vi "MecaKinematics_ToChassisSpeeds.vi"(9 "MECA_WHEEL_SPEEDS":T4 {"RearRightSpeed" format="%19.3f"; "RearLeftSpeed" format="%19.3f"; "FrontRightSpeed" format="%19.3f"; "FrontLeftSpeed" format="%19.3f"}, 11 "in MECA_DRIVE_KINEMATICS":T1={"FrontLeft"={"X"=0.0, "Y"=0.0}, "FrontRight"={"X"=0.0, "Y"=0.0}, "RearLeft"={"X"=0.0, "Y"=0.0}, "RearRight"={"X"=0.0, "Y"=0.0}, "InverseKinematics"=[[0.0, 1.0, -1.0, 0.0], [0.0, 1.0, 1.0, 0.0], [0.0, 1.0, 1.0, 0.0], [0.0, 1.0, -1.0, 0.0]], "ForwardKinematics"=[[0.0, 1.0, -1.0, 0.0], [0.0, 1.0, 1.0, 0.0], [0.0, 1.0, 1.0, 0.0], [0.0, 1.0, -1.0, 0.0]], "PrevCoR"={"X"=0.0, "Y"=0.0}} {"PrevCoR"."Y" format="%14.3f"; "PrevCoR"."X" format="%14.3f"; "RearRight"."Y" format="%14.3f"; "RearRight"."X" format="%14.3f"; "RearLeft"."Y" format="%14.3f"; "RearLeft"."X" format="%14.3f"; "FrontRight"."Y" format="%14.3f"; "FrontRight"."X" format="%14.3f"; "FrontLeft"."Y" format="%14.3f"; "FrontLeft"."X" format="%14.3f"}) -> (3 "ChassisSpeeds":T5 {"vOmega" format="%10.3f"; "vY" format="%10.3f"; "vX" format="%10.3f"})   [LabVIEW 2019, in "Trajectory_Library.lvlib"]
doc: "Performs forward kinematics to return the resulting chassis state from the given wheel speeds. This method is often used for odometry -- determining the robot's position on the field using data from the real-world speed of each wheel on the robot.\n\nParametetrs:\n - MecaDriveKinematics - Data structure\n - WheelSpeeds - The current mecanum drive wheel speeds.\n\nReturns:\n - ChassisSpeeds - The resulting chassis speed."
uses:
  Trajectory_Library.lvlib
  <vilib>/Analysis/Matrix/NI_Matrix.lvlib
  <vilib>/Analysis/Matrix/Numeric/Multiply/Multiply - RM,RM.vi
  TypeDef/TRANSLATION2D.ctl
  TypeDef/CHASSIS_SPEEDS.ctl
  TypeDef/MECA_WHEEL_SPEEDS.ctl
  <vilib>/Analysis/Matrix/Datatypes/RealMatrix.ctl
  TypeDef/MECA_DRIVE_KINEMATICS.ctl
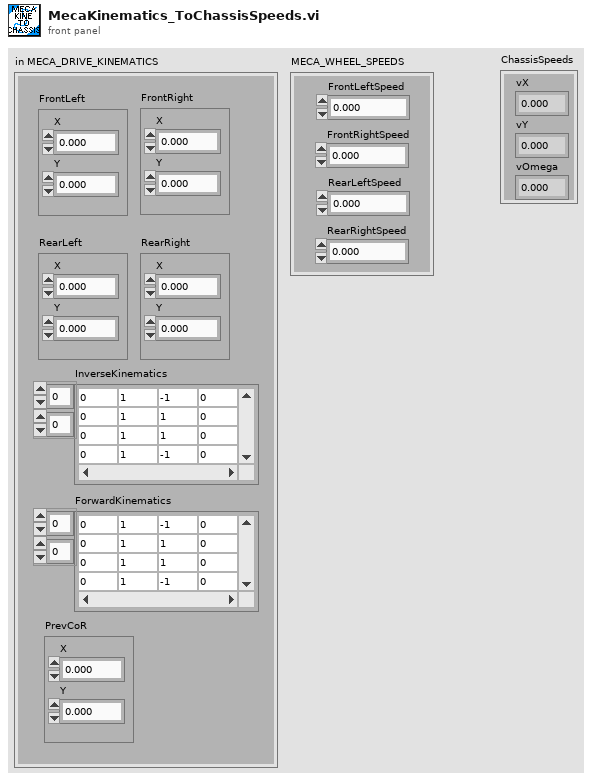
[diagram p1: front panel]
types:
  T1 = typedef "Trajectory_Library.lvlib/MECA_DRIVE_KINEMATICS.ctl" = cluster{"FrontLeft":T2, "FrontRight":T2, "RearLeft":T2, "RearRight":T2, "InverseKinematics":T3, "ForwardKinematics":T3, "PrevCoR":T2}
  T2 = typedef "Trajectory_Library.lvlib/TRANSLATION2D.ctl" = cluster{"X":dbl, "Y":dbl}
  T3 = typedef "NI_Matrix.lvlib/RealMatrix.ctl" = dbl[][]
  T4 = typedef "Trajectory_Library.lvlib/MECA_WHEEL_SPEEDS.ctl" = cluster{"FrontLeftSpeed":dbl, "FrontRightSpeed":dbl, "RearLeftSpeed":dbl, "RearRightSpeed":dbl}
  T5 = typedef "Trajectory_Library.lvlib/CHASSIS_SPEEDS.ctl" = cluster{"vX":dbl, "vY":dbl, "vOmega":dbl}
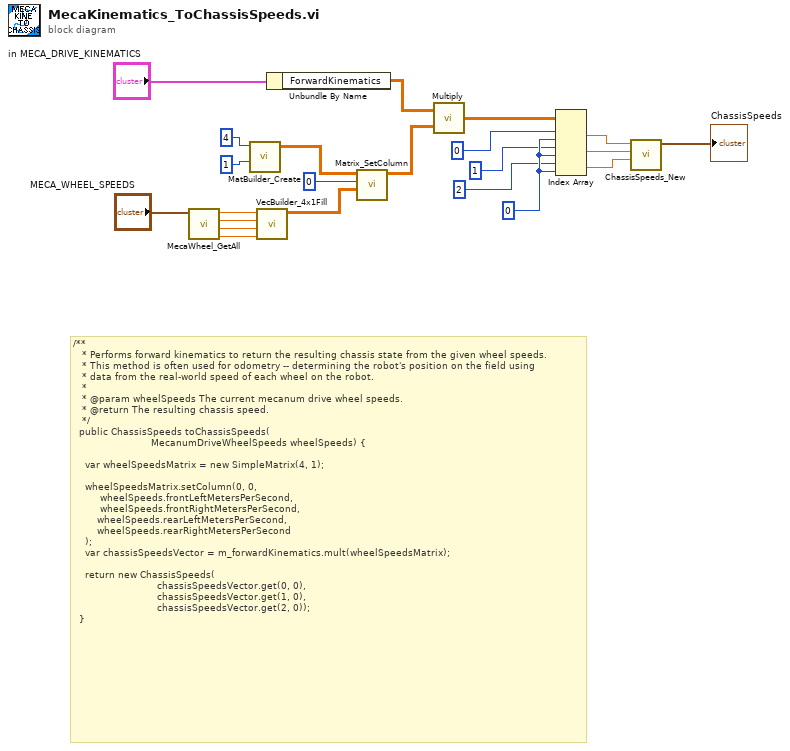
[diagram p0: block diagram]
diagram:
  w22 = 0 ("index (col)")
  # "/**\n   * Performs forward kinematics to return the resulting chassis state from the given wheel speeds.\n   * This method is often used for odometry -- determining the robot's position on the field using\n   * data from the real-world speed of each wheel on the robot.\n   *\n   * @param wheelSpeeds The current mecanum drive wheel speeds.\n   * @return The resulting chassis speed.\n   */\n  public ChassisSpeeds toChassisSpeeds(\n                          MecanumDriveWheelSpeeds wheelSpeeds) {\n\n    var wheelSpeedsMatrix = new SimpleMatrix(4, 1);\n\n    wheelSpeedsMatrix.setColumn(0, 0,\n         wheelSpeeds.frontLeftMetersPerSecond, \n         wheelSpeeds.frontRightMetersPerSecond,\n        wheelSpeeds.rearLeftMetersPerSecond, \n        wheelSpeeds.rearRightMetersPerSecond\n    );\n    var chassisSpeedsVector = m_forwardKinematics.mult(wheelSpeedsMatrix);\n\n    return new ChassisSpeeds(\n                            chassisSpeedsVector.get(0, 0), \n                            chassisSpeedsVector.get(1, 0),\n                            chassisSpeedsVector.get(2, 0));\n  }"
  n1 = call "MecaWheel_GetAll.vi"("MECA_WHEEL_SPEEDS"="MECA_WHEEL_SPEEDS") -> ("RearRightSpeed"=w1:dbl, "RearLeftSpeed"=w2:dbl, "FrontRightSpeed"=w3:dbl, "FrontLeftSpeed"=w4:dbl)  [unwired: 7 in]
  n2 = call "MatBuilder_Create.vi"("Columns"=1, "Rows"=4) -> ("output matrix"=w9:T3)  [unwired: 9 in]
  n3 = call "VecBuilder_4x1Fill.vi"("R3"=w1, "R2"=w2, "R1"=w3, "R0"=w4) -> ("output matrix"=w7:T3)  [unwired: 7 in]
  n4 = Unbundle By Name("in MECA_DRIVE_KINEMATICS") -> ("ForwardKinematics"=w17:T3)
  n5 = call "Matrix_SetColumn.vi"("Fill Vector"=w7, "Column"=0, "input matrix"=w9) -> ("output matrix"=w6:T3)  [unwired: 7 in, 1 out]
  n6 = call-poly <vilib>:"Multiply.vi"("Real Matrix B"=w6, "Real Matrix A"=w17) -> ("A * B"=w16:T3)
  n7 = Index Array(array=w16, index (row) #1=0 ("index (row)"), index (col) #1=w22, index (row) #2=1 ("index (row)"), index (col) #2=w22, index (row) #3=2 ("index (row)"), index (col) #3=w22) -> (element #1=w15:dbl, element #2=w14:dbl, element #3=w13:dbl)
  n8 = call "ChassisSpeeds_New.vi"("vAngular"=w13, "vY"=w14, "vX"=w15) -> ("CHASSIS"=→"ChassisSpeeds":T5)  [unwired: 8 in]
